vi "Evaluate All Checks.vi"(8 "error in":errorcluster, 9 "checks":T1, 10 "bool values":cluster{"name":string, "on":bool}[](array[cluster]), 11 "num values":cluster{"channel":string, "value":dbl}[](array[cluster])) -> (0 "error out":errorcluster, 2 "first fail":string, 3 "passes":bool)   [LabVIEW 2026]
doc: "Aggregate over all check sections in documented order: di_high, di_low, misc_high, misc_low, t0_high, t0_low, misc_compare. Every configured section must pass; the name of the first failing item (earliest section first) is reported. Anything not configured passes."
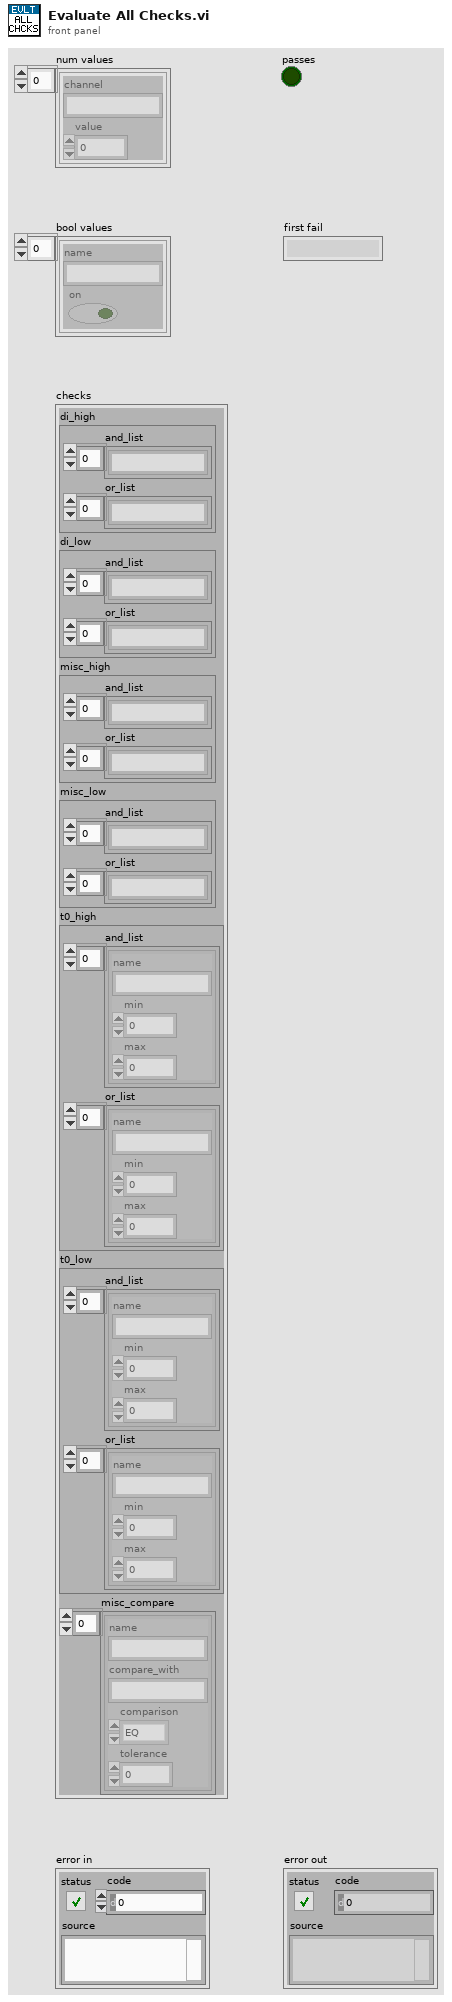
[diagram p1: front panel]
types:
  T1 = cluster{"di_high":cluster{"and_list":string[], "or_list":string[]}, "di_low":cluster{"and_list":string[], "or_list":string[]}, "misc_high":cluster{"and_list":string[], "or_list":string[]}, "misc_low":cluster{"and_list":string[], "or_list":string[]}, "t0_high":cluster{"and_list":cluster{"name":string, "min":dbl, "max":dbl}[], "or_list":cluster{"name":string, "min":dbl, "max":dbl}[]}, "t0_low":cluster{"and_list":cluster{"name":string, "min":dbl, "max":dbl}[], "or_list":cluster{"name":string, "min":dbl, "max":dbl}[]}, "misc_compare":cluster{"name":string, "compare_with":string, "comparison":enum16{"EQ", "NE", "GT", "GE", "LT", "LE"}, "tolerance":dbl}[]}
  T2 = cluster{"and_list":cluster{"name":string, "min":dbl, "max":dbl}[], "or_list":cluster{"name":string, "min":dbl, "max":dbl}[]}
  T3 = cluster{"name":string, "compare_with":string, "comparison":enum16{"EQ", "NE", "GT", "GE", "LT", "LE"}, "tolerance":dbl}[]
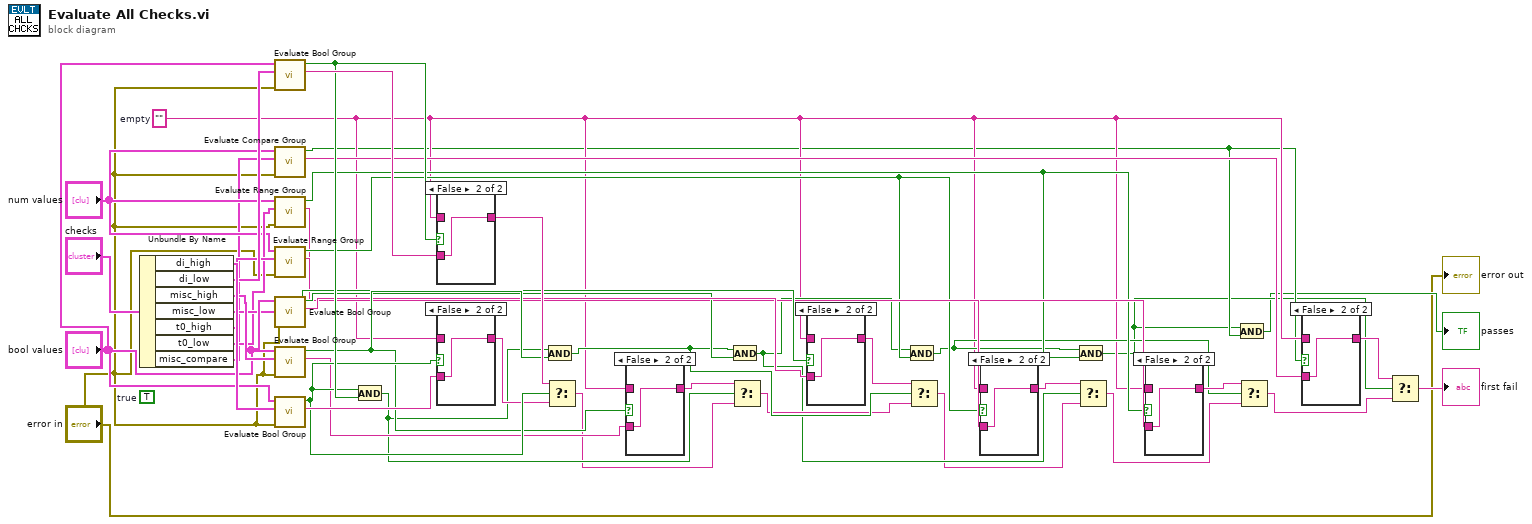
[diagram p0: block diagram]
diagram:
  w8 = ""  # empty
  (unwired) TRUE  # true
  n1 = Unbundle By Name("checks") -> ("di_high"=w44:cluster{"and_list":string[], "or_list":string[]}, "di_low"=w42:cluster{"and_list":string[], "or_list":string[]}, "misc_high"=w36:cluster{"and_list":string[], "or_list":string[]}, "misc_low"=w29:cluster{"and_list":string[], "or_list":string[]}, "t0_high"=w23:T2, "t0_low"=w17:T2, "misc_compare"=w10:T3)
  n2 = call "Evaluate Bool Group.vi"("error in"="error in", "group"=w42, "bool values"="bool values") -> ("first fail"=w41:string, "passes"=w40:bool)  [unwired: 6 in, 1 out]
  n3 = call "Evaluate Compare Group.vi"("error in"="error in", "items"=w10, "num values"="num values") -> ("first fail"=w9:string, "passes"=w7:bool)  [unwired: 6 in, 1 out]
  n4 = call "Evaluate Range Group.vi"("error in"="error in", "group"=w17, "num values"="num values") -> ("first fail"=w16:string, "passes"=w15:bool)  [unwired: 6 in, 1 out]
  n5 = call "Evaluate Range Group.vi"("error in"="error in", "group"=w23, "num values"="num values") -> ("first fail"=w22:string, "passes"=w21:bool)  [unwired: 6 in, 1 out]
  n6 = call "Evaluate Bool Group.vi"("error in"="error in", "group"=w29, "bool values"="bool values") -> ("first fail"=w28:string, "passes"=w27:bool)  [unwired: 6 in, 1 out]
  n7 = call "Evaluate Bool Group.vi"("error in"="error in", "group"=w36, "bool values"="bool values") -> ("first fail"=w35:string, "passes"=w34:bool)  [unwired: 6 in, 1 out]
  n8 = call "Evaluate Bool Group.vi"("error in"="error in", "group"=w44, "bool values"="bool values") -> ("first fail"=w43:string, "passes"=w38:bool)  [unwired: 6 in, 1 out]
  n9 = And(x=w38, y=w40) -> (x .and. y?=w32:bool)
  n10 = case shown="False" w40 {
    tunnel: w41 -> [_ w47]
    tunnel: [w46 w47] -> w39
    tunnel: w8 -> [w46 _]
    frame True {
    }
    frame False {
    }
  }
  n11 = case shown="False" w38 {
    tunnel: w43 -> [_ w49]
    tunnel: [w48 w49] -> w37
    tunnel: w8 -> [w48 _]
    frame True {
    }
    frame False {
    }
  }
  n12 = And(x=w32, y=w34) -> (x .and. y?=w25:bool)
  n13 = Select(t=w39, s=w38, f=w37) -> (s? t:f=w31:string)
  n14 = case shown="False" w34 {
    tunnel: w35 -> [_ w51]
    tunnel: [w50 w51] -> w33
    tunnel: w8 -> [w50 _]
    frame True {
    }
    frame False {
    }
  }
  n15 = And(x=w25, y=w27) -> (x .and. y?=w19:bool)
  n16 = Select(t=w33, s=w32, f=w31) -> (s? t:f=w24:string)
  n17 = case shown="False" w27 {
    tunnel: w28 -> [_ w53]
    tunnel: [w52 w53] -> w26
    tunnel: w8 -> [w52 _]
    frame True {
    }
    frame False {
    }
  }
  n18 = And(x=w19, y=w21) -> (x .and. y?=w13:bool)
  n19 = Select(t=w26, s=w25, f=w24) -> (s? t:f=w18:string)
  n20 = case shown="False" w21 {
    tunnel: w22 -> [_ w55]
    tunnel: [w54 w55] -> w20
    tunnel: w8 -> [w54 _]
    frame True {
    }
    frame False {
    }
  }
  n21 = And(x=w13, y=w15) -> (x .and. y?=w5:bool)
  n22 = Select(t=w20, s=w19, f=w18) -> (s? t:f=w12:string)
  n23 = case shown="False" w15 {
    tunnel: w16 -> [_ w57]
    tunnel: [w56 w57] -> w14
    tunnel: w8 -> [w56 _]
    frame True {
    }
    frame False {
    }
  }
  n24 = And(x=w5, y=w7) -> (x .and. y?=→"passes":bool)
  n25 = Select(t=w14, s=w13, f=w12) -> (s? t:f=w4:string)
  n26 = case shown="False" w7 {
    tunnel: w9 -> [_ w59]
    tunnel: [w58 w59] -> w6
    tunnel: w8 -> [w58 _]
    frame True {
    }
    frame False {
    }
  }
  n27 = Select(t=w6, s=w5, f=w4) -> (s? t:f=→"first fail":string)
  "error out" <- "error in"
